vi "xnet_canopen_bind_batch.vi"(8 "error in (no error)":errorcluster, 10 "OD Indices":T1[](array[typedef]) {"SubIndex" format="%.0x"; "Index" format="%.0x"}, 11 "xnet_co_handle_in":u64) -> (0 "error out":errorcluster, 2 "OD Batch":refnum<class "OD Batch.lvclass">, 3 "xnet_co_handle":u64)   [LabVIEW 2023, in "xnet_canopen.lvlib"]
uses:
  xnet_canopen.lvlib
  typedef/od index.ctl
  OD Batch/OD Batch.lvclass
  typedef/od entry.ctl
  typedef/canopen types.ctl
  <vilib>/Utility/error.llb/Error Cluster From Error Code.vi
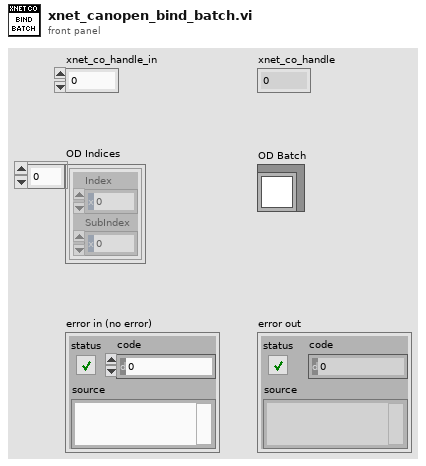
[diagram p1: front panel]
types:
  T1 = typedef "xnet_canopen.lvlib/od index.ctl" = cluster{"Index":u16, "SubIndex":u8}
  T2 = typedef "xnet_canopen.lvlib/od entry.ctl" = cluster{"OD Index":T1, "CANOpen Types":T3, "Size":u32, "Offset":u32, "Value":variant, "Initialized":bool}
  T3 = typedef "xnet_canopen.lvlib/canopen types.ctl" = u32
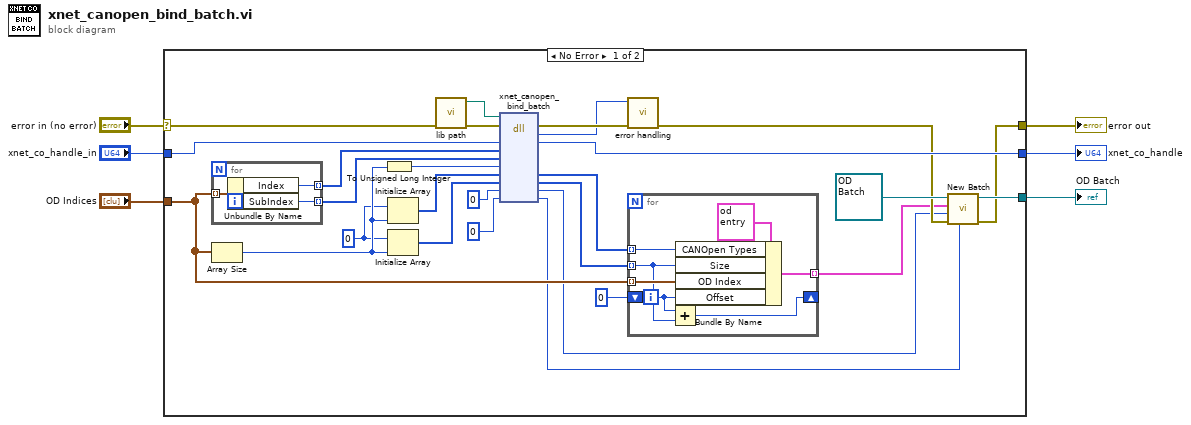
[diagram p0: block diagram]
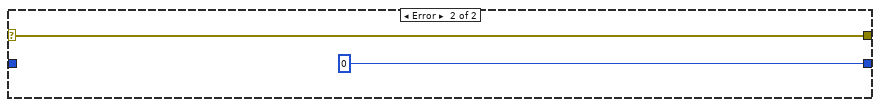
[diagram p2: hidden frame]
diagram:
  n1 = case shown="No Error" "error in (no error)" {
    selector: "error in (no error)" -> [w31 w44]
    tunnel: [w8 w44] -> w5
    tunnel: [w28 u64 0 ("phandle")] -> w4
    tunnel: "xnet_co_handle_in" -> [w27 _]
    tunnel: "OD Indices" -> [w15 _]
    tunnel: [w9 _] -> w1
    frame No Error {
      w20 = u32 0 ("element")
      n2 = for {
        tunnel: w15 -> [w42] mode=indexing
        tunnel: [w41] -> w26 mode=indexing
        tunnel: [w40] -> w25 mode=indexing
        n3 = Unbundle By Name(w42) -> ("Index"=w41:u16, "SubIndex"=w40:u8)
      }
      n4 = Array Size(array=w15) -> (size(s)=w23:i32)
      n5 = To Unsigned Long Integer(number=w23) -> (unsigned 32bit integer=w24:u32)
      n6 = Initialize Array(w20, w23) -> (w22:u32[])
      n7 = Initialize Array(w20, w23) -> (w21:u32[])
      n8 = call "lib path.vi"() -> ("lib path"=w32:path)  [unwired: 11 in]
      n9 = dll-call lib="?" fn="xnet_canopen_bind_batch"(path in=w32, error in=w31, "handle"=w27, "indices"=w26, "subindices"=w25, "count"=w24, "types"=w22, "val_sizes"=w21, "bufsize"=u32 0, "batch_id"=u32 0) -> (error out=w30:errorcluster, "return type"=w29:i32, "handle"=w28:u64, "types"=w17:u32[], "val_sizes"=w16:u32[], "bufsize"=w11:u32, "batch_id"=w10:u32)  [unwired: 4 in, 1 out]
      n10 = call "error handling.vi"("error in (no error)"=w30, "return val"=w29) -> ("error out"=w13:errorcluster)  [unwired: 9 in]
      n11 = for {
        tunnel: w17 -> [w38] mode=indexing
        tunnel: w16 -> [w34] mode=indexing
        tunnel: w15 -> [w37] mode=indexing
        tunnel: [w36] -> w12 mode=indexing
        shift-right: [w33] -> _
        shift-left: u32 0 ("Offset") -> [w35]
        n12 = Add(x=w35, y=w34) -> (x+y=w33:u32)
        n13 = Bundle By Name(cluster=T2 {"OD Index"={"Index"=0, "SubIndex"=0}, "CANOpen Types"=0, "Size"=0, "Offset"=0, "Value"=variant, "Initialized"=FALSE} ("OD Entry"), "CANOpen Types"=w38, "Size"=w34, "OD Index"=w37, "Offset"=w35) -> (w36:T2)
      }
      n14 = call "New Batch.vi"("Batch ID"=w10, "error in (no error)"=w13, "Buffer size"=w11, "OD Vars"=w12, "OD Batch in"=refnum<class "OD Batch.lvclass"> refnum ("OD Batch")) -> ("error out"=w8:errorcluster, "OD Batch out"=w9:refnum<class "OD Batch.lvclass">)  [unwired: 5 in]
    }
    frame Error {
    }
  }
  "error out" <- w5
  "xnet_co_handle" <- w4
  "OD Batch" <- w1
